vi "GetTemplatePath.vi"(0 "reference in":refnum<class "ClassWriterGOOP300.lvclass">, 1 "ClassTemplateSubDirectory":string, 5 "error in (no error)":errorcluster) -> (14 "reference out":refnum<class "ClassWriterGOOP300.lvclass">, 15 "FolderPathOut":path, 17 "MethodTemplatePathOut":path, 18 "TemplateSettings":T1, 19 "error out":errorcluster)   [LabVIEW 2020, in "ClassWriterGOOP300.lvclass"]
uses:
  <resource>/Framework/Providers/Open_GDS/ClassProviders/Provider_EndevoGOOP300/ClassWriterGOOP300_class/ClassWriterGOOP300.lvclass
  <resource>/Framework/Providers/Open_GDS/ClassProviders/Provider_BaseClassInterface/ClassWriter_class/TemplateSettings.ctl
  <resource>/Framework/Providers/Open_GDS/ClassProviders/Provider_EndevoGOOP300/ClassWriterGOOP300_class/ClassWriterGOOP300.lvclass/ClassWriterGOOP300.ctl
  <resource>/Framework/Providers/Open_GDS/ClassProviders/Provider_LvNativeClass/ClassWriterNative_class/ClassWriterNative.lvclass
  C:/Program Files (x86)/National Instruments/LabVIEW 2020/resource/Framework/Providers/Open_GDS/ClassProviders/Provider_LvNativeClass/ClassWriterNative_class/ClassWriterNative.lvclass
  C:/Program Files (x86)/National Instruments/LabVIEW 2020/resource/Framework/Providers/Open_GDS/ClassProviders/Provider_BaseClassInterface/ClassWriter_class/ClassWriter.lvclass
  C:/Program Files (x86)/National Instruments/LabVIEW 2020/resource/Framework/Providers/Open_GDS/ClassProviders/Provider_EndevoGOOP300/ClassWriterGOOP300_class/ClassWriterGOOP300.lvclass
  <resource>/Framework/Providers/Open_GDS/ClassProviders/Provider_BaseClassInterface/ClassWriter_class/ClassWriter.lvclass
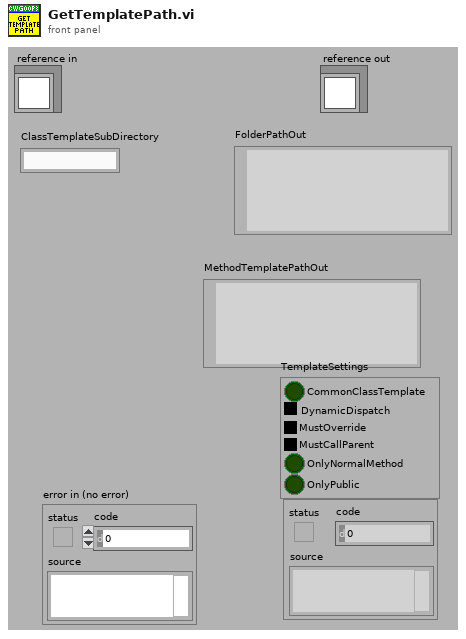
[diagram p1: front panel]
types:
  T1 = typedef "ClassWriter.lvclass/TemplateSettings.ctl" = cluster{"CommonClassTemplate":bool, "DynamicDispatch":enum8{"False", "True", "Mixed"}, "MustOverride":enum8{"False", "True", "Mixed"}, "MustCallParent":enum8{"False", "True", "Mixed"}, "OnlyNormalMethod":bool, "OnlyPublic":bool}
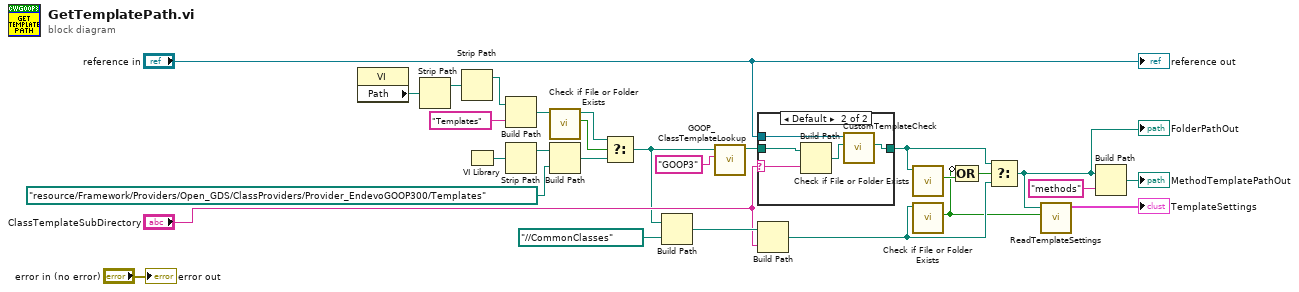
[diagram p0: block diagram]
diagram:
  n1 = property class="VI"() -> ("Path"=w26:path)  [unwired: 2 in, 2 out]
  n2 = Strip Path(path=w26) -> (stripped path=w24:path)  [unwired: 1 out]
  n3 = Strip Path(path=w24) -> (stripped path=w28:path)  [unwired: 1 out]
  n4 = VI Library() -> (path=w20:path)
  n5 = Build Path(base path=w28, name or relative path="Templates") -> (appended path=w21:path)
  n6 = Strip Path(path=w20) -> (stripped path=w15:path)  [unwired: 1 out]
  n7 = call <vilib>:"Check if File or Folder Exists.vi"("path"=w21) -> ("file or folder exists?"=w23:bool, "dup path"=w22:path)  [unwired: 8 in, 1 out]
  n8 = Build Path(base path=w15, name or relative path=path "resource/Framework/Providers/Open_GDS/ClassProviders/Provider_EndevoGOOP300/Templates" ("base path")) -> (appended path=w18:path)
  n9 = Select(t=w22, s=w23, f=w18) -> (s? t:f=w8:path)
  n10 = Build Path(base path=w8, name or relative path=path "../../CommonClasses") -> (appended path=w10:path)
  n11 = call <resource>:"GOOP_ClassTemplateLookup.vi"("ClassType"="GOOP3", "ClassTemplateFolderIn"=w8) -> ("ClassTemplateFolderOut"=w13:path)  [unwired: 9 in]
  n12 = case shown="Default" "ClassTemplateSubDirectory" {
    selector: "ClassTemplateSubDirectory" -> [_ w33]
    tunnel: w13 -> [w29 w34]
    tunnel: [w29 w30] -> w12
    tunnel: "reference in" -> [_ w31]
    frame "" {
    }
    frame Default {
      n13 = Build Path(base path=w34, name or relative path=w33) -> (appended path=w32:path)
      n14 = call <resource>:"CustomTemplateCheck.vi"("ClassTemplate"=w32, "ClassWriterNative in"=w31) -> ("ClassTemplate(Maybe Modified if not exists)"=w30:path)  [unwired: 9 in]
    }
  }
  n15 = Build Path(base path=w10, name or relative path="ClassTemplateSubDirectory") -> (appended path=w5:path)
  n16 = call <vilib>:"Check if File or Folder Exists.vi"("path"=w12) -> ("file or folder exists?"=w4:bool)  [unwired: 8 in, 2 out]
  n17 = call <vilib>:"Check if File or Folder Exists.vi"("path"=w5) -> ("file or folder exists?"=w2:bool)  [unwired: 8 in, 2 out]
  n18 = Compound Arithmetic op=OR(invert w2, w4) -> (w3:bool)
  n19 = Select(t=w12, s=w3, f=w5) -> (s? t:f=w6:path)
  "FolderPathOut" <- w6
  n20 = call <resource>:"ReadTemplateSettings.vi"("CommonClassTemplate"=w2, "TemplateFolder"=w6) -> ("TemplateSettings"=→"TemplateSettings":T1)  [unwired: 9 in]
  n21 = Build Path(base path=w6, name or relative path="methods") -> (appended path=→"MethodTemplatePathOut":path)
  "error out" <- "error in (no error)"
  "reference out" <- "reference in"
